vi "UpdateNativePropertyMethod.vi"(1 "VI":refnum<vi>, 2 "TypeDefControl":path=path "C:/classes/ObjectAttributes.ctl", 3 "Property":string, 5 "error IO":errorcluster, 6 "GetMethod":bool) -> (19 "error out":errorcluster)   [LabVIEW 2020, in "ClassWriterNative.lvclass"]
uses:
  ClassWriterNative.lvclass
  <vilib>/Utility/miscctls.llb/LVPositionTypeDef.ctl
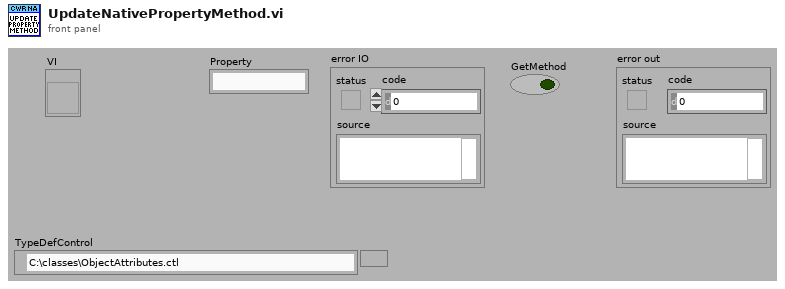
[diagram p1: front panel]
types:
  T1 = typedef "LVPositionTypeDef.ctl" = cluster{"Left":i32, "Top":i32}
  T2 = enum16{"Invalid Wire Rule", "Required", "Recommended", "Optional", "Dynamic Dispatch"}
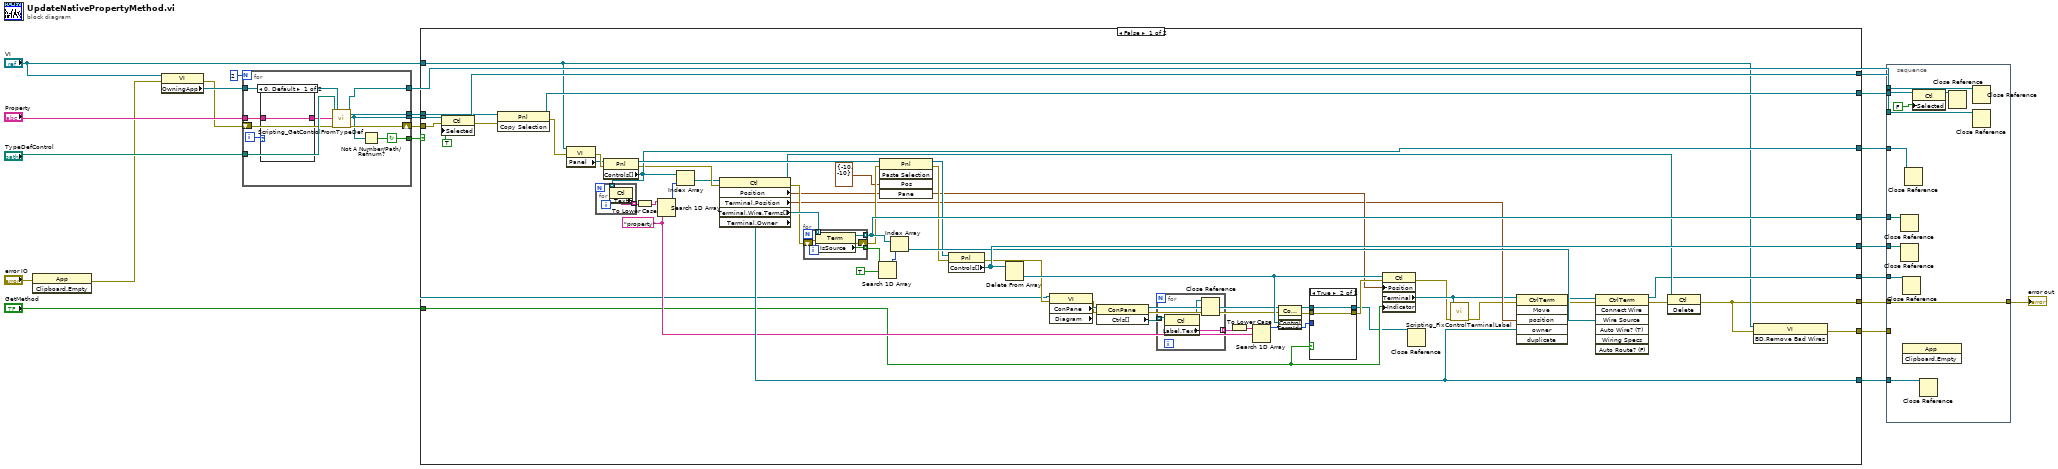
[diagram p0: block diagram]
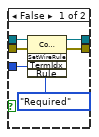
[diagram p2: hidden frame]
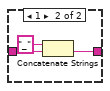
[diagram p4: hidden frame]
diagram:
  n1 = invoke class="App" method="Clipboard.Empty"(error in="error IO") -> (error out=w8:errorcluster)  [unwired: 2 in, 2 out]
  n2 = property class="VI"(reference="VI", error in=w8) -> (error out=w7:errorcluster, "OwningApp"=w9:refnum<vi>)  [unwired: 1 out]
  n3 = for {
    N: 2 -> [_]
    tunnel: [w29] -> w17
    tunnel: "Property" -> [w27]
    tunnel: [w34] -> w2
    tunnel: [w33] -> w13
    tunnel: "TypeDefControl" -> [w32]
    tunnel: w9 -> [w31]
    shift-right: [w35] -> w18
    shift-left: w7 -> [w30]
    tunnel: [w25] -> w1
    i -> [w28]
    stop <- w25 continue-if-true
    n4 = case shown="0, Default" w28 {
      tunnel: w27 -> [w36 w39]
      tunnel: [w36 w37] -> w26
      frame 0, Default {
      }
      frame 1 {
        n5 = Concatenate Strings("_" ("string"), w39) -> (w37:string)
      }
    }
    n6 = call "Scripting_GetControlFromTypeDef.vi"("TypeDefControl"=w32, "String"=w26, "error in"=w30, "AppRef"=w31) -> ("vi reference"=w34:refnum<vi>, "Panel"=w33:refnum<vi>, "ControlRef"=w29:refnum<vi>, "error out"=w35:errorcluster)  [unwired: 12 in]
    n7 = Not A Number/Path/Refnum?(number/path/refnum=w29) -> (NaN/Path/Refnum?=w25:bool)
  }
  n8 = case shown="False" w1 {
    tunnel: [w93 _] -> w24
    tunnel: [w92 _] -> w23
    tunnel: [w91 _] -> w22
    tunnel: [w90 _] -> w21
    tunnel: [w89 _] -> w20
    tunnel: w18 -> [w75 w117]
    tunnel: w17 -> [w73 _]
    tunnel: [w62 _] -> w15
    tunnel: [w60 _] -> w14
    tunnel: w13 -> [w59 _]
    tunnel: "GetMethod" -> [w51 _]
    tunnel: "VI" -> [w47 _]
    tunnel: [w46 w117] -> w5
    tunnel: [w45 _] -> w4
    frame False {
      w56 = "property" ("element")
      n9 = property class="Ctl"(reference=w73, error in=w75, "Selected"=TRUE) -> (reference out=w90:refnum<vi>, error out=w74:errorcluster)
      n10 = invoke class="Pnl" method="Copy Selection"(reference=w59, error in=w74) -> (reference out=w89:refnum<vi>, error out=w76:errorcluster)  [unwired: 1 in, 1 out]
      n11 = property class="VI"(reference=w47, error in=w76) -> (error out=w78:errorcluster, "Panel"=w77:refnum<vi>)  [unwired: 1 out]
      n12 = property class="Pnl"(reference=w77, error in=w78) -> (reference out=w95:refnum<vi>, error out=w82:errorcluster, "Controls[]"=w91:refnum<vi>[])
      n13 = for {
        tunnel: w91 -> [w116] mode=indexing
        tunnel: [w115] -> w79 mode=indexing
        n14 = property class="Ctl"(reference=w116) -> ("Label.Text"=w115:string)  [unwired: 1 in, 2 out]
      }
      n15 = To Lower Case(string=w79) -> (all lower case string=w94:string[])
      n16 = Search 1D Array(1D array=w94, element=w56) -> (index of element=w80:i32)  [unwired: 1 in]
      n17 = Index Array(array=w91, index=w80) -> (element=w81:refnum<vi>)
      n18 = property class="Ctl"(reference=w81, error in=w82) -> (reference out=w68:refnum<vi>, error out=w71:errorcluster, "Position"=w63:T1, "Terminal.Position"=w61:T1, "Terminal.Wire.Terms[]"=w83:refnum<vi>[], "Terminal.Owner"=w60:refnum<vi>)
      n19 = for {
        tunnel: w83 -> [w114] mode=indexing
        tunnel: [w113] -> w84 mode=indexing
        tunnel: [w112] -> w92 mode=indexing
        shift-right: [w110] -> w70
        shift-left: w71 -> [w111]
        n20 = property class="Term"(reference=w114, error in=w111) -> (reference out=w112:refnum<vi>, error out=w110:errorcluster, "IsSource"=w113:bool)
      }
      n21 = Search 1D Array(1D array=w84, element=TRUE) -> (index of element=w86:i32)  [unwired: 1 in]
      n22 = invoke class="Pnl" method="Paste Selection"(reference=w95, error in=w70, "Pos"=T1 {"Left"=-10, "Top"=-10} ("Position")) -> (reference out=w87:refnum<vi>, error out=w67:errorcluster)  [unwired: 2 in, 3 out]
      n23 = Index Array(array=w92, index=w86) -> (element=w88:refnum<vi>)
      n24 = property class="Pnl"(reference=w87, error in=w67) -> (error out=w66:errorcluster, "Controls[]"=w93:refnum<vi>[])  [unwired: 1 out]
      n25 = Delete From Array(array=w93) -> (deleted portion=w96:refnum<vi>)  [unwired: 2 in, 1 out]
      n26 = property class="VI" props=["ConPane", "Diagram"](reference=w47, error in=w66) -> (error out=w49:errorcluster, "ConPane"=w58:refnum<vi>)  [unwired: 2 out]
      n27 = property class="ConPane"(reference=w58, error in=w49) -> (reference out=w53:refnum<vi>, error out=w52:errorcluster, "Ctrls[]"=w57:refnum<vi>[])
      n28 = for {
        tunnel: w57 -> [w100] mode=indexing
        tunnel: [w101] -> w55 mode=indexing
        n29 = property class="Ctl"(reference=w100) -> (reference out=w99:refnum<vi>, "Label.Text"=w101:string)  [unwired: 1 in, 1 out]
        n30 = Close Reference(reference=w99) -> ()  [unwired: 1 in, 1 out]
      }
      n31 = To Lower Case(string=w55) -> (all lower case string=w54:string[])
      n32 = Search 1D Array(1D array=w54, element=w56) -> (index of element=w50:i32)  [unwired: 1 in]
      n33 = invoke class="ConPane" method="AssignCtrlToTerm"(reference=w53, error in=w52, "Control"=w96, "TermIdx"=w50) -> (reference out=w97:refnum<vi>, error out=w98:errorcluster)  [unwired: 1 in, 3 out]
      n34 = case shown="True" w51 {
        tunnel: w97 -> [w107 w108]
        tunnel: w98 -> [w106 w109]
        tunnel: [w104 w109] -> w64
        tunnel: w50 -> [w103 _]
        tunnel: [w102 w108] -> w48
        frame False {
          n35 = invoke class="ConPane" method="SetWireRule"(reference=w107, error in=w106, "TermIdx"=w103, "Rule"=T2."Required") -> (reference out=w102:refnum<vi>, error out=w104:errorcluster)  [unwired: 1 in, 3 out]
        }
        frame True {
        }
      }
      n36 = property class="Ctl"(reference=w96, error in=w64, "Position"=w63, "Indicator"=w51) -> (error out=w41:errorcluster, "Terminal"=w42:refnum<vi>)  [unwired: 1 out]
      n37 = Close Reference(reference=w48) -> ()  [unwired: 1 in, 1 out]
      n38 = call "Scripting_FixControlTerminalLabel.vi"("error in (no error)"=w41, "ControlTerminalRef"=w42) -> ("error out"=w40:errorcluster)  [unwired: 8 in, 1 out]
      n39 = invoke class="CtrlTerm" method="Move"(reference=w42, error in=w40, "position"=w61, "owner"=w60) -> (reference out=w44:refnum<vi>, error out=w43:errorcluster)  [unwired: 2 in, 4 out]
      n40 = invoke class="CtrlTerm" method="Connect Wire"(reference=w44, error in=w43, "Wire Source"=w88) -> (reference out=w62:refnum<vi>, error out=w69:errorcluster)  [unwired: 4 in, 5 out]
      n41 = invoke class="Ctl" method="Delete"(reference=w68, error in=w69) -> (error out=w46:errorcluster)  [unwired: 1 in, 2 out]
      n42 = invoke class="VI" method="BD.Remove Bad Wires"(reference=w47, error in=w46) -> (error out=w45:errorcluster)  [unwired: 1 in, 2 out]
    }
    frame True {
    }
  }
  n43 = stacked-sequence {
    tunnel: w5 -> [w128]
    tunnel: [w128] -> w19
    tunnel: w2 -> [w127]
    tunnel: w20 -> [w126]
    tunnel: w21 -> [w122]
    tunnel: w22 -> [w120]
    tunnel: w23 -> [w119]
    tunnel: w24 -> [w118]
    tunnel: w15 -> [w125]
    tunnel: w14 -> [w124]
    tunnel: w4 -> [_]
    frame #0 {
      n44 = Close Reference(reference=w119) -> ()  [unwired: 1 in, 1 out]
      n45 = Close Reference(reference=w118) -> ()  [unwired: 1 in, 1 out]
      n46 = Close Reference(reference=w125) -> ()  [unwired: 1 in, 1 out]
      n47 = invoke class="App" method="Clipboard.Empty"() -> ()  [unwired: 3 in, 3 out]
      n48 = Close Reference(reference=w120) -> ()  [unwired: 1 in, 1 out]
      n49 = property class="Ctl"(reference=w122, "Selected"=FALSE) -> (reference out=w121:refnum<vi>)  [unwired: 1 in, 1 out]
      n50 = Close Reference(reference=w124) -> ()  [unwired: 1 in, 1 out]
      n51 = Close Reference(reference=w121) -> ()  [unwired: 1 in, 1 out]
      n52 = Close Reference(reference=w127) -> ()  [unwired: 1 in, 1 out]
      n53 = Close Reference(reference=w126) -> ()  [unwired: 1 in, 1 out]
    }
  }
  "error out" <- w19
